vi "rename tag writer or reader.vi"(6 "new channel":refnum<class "TBM channel.lvclass">, 7 "owner ID":string, 8 "error in":errorcluster, 9 "old channel":refnum<class "TBM channel.lvclass">, 10 "tag descriptor":refnum<class "tag descriptor.lvclass">, 11 "engine configuration in":refnum<class "engine configuration.lvclass">) -> (0 "error out":errorcluster, 3 "engine configuration out":refnum<class "engine configuration.lvclass">)   [LabVIEW 2014, in "engine configuration.lvclass"]
uses:
  engine configuration.lvclass
  <vilib>/NI/Tag Bus/tag/tag descriptor.lvclass
  <vilib>/NI/Tag Bus Module Framework/channel/TBM channel.lvclass
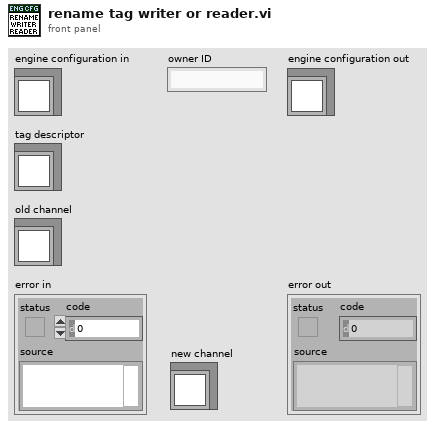
[diagram p1: front panel]
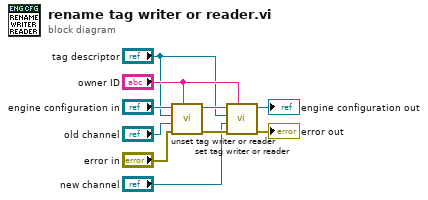
[diagram p0: block diagram]
diagram:
  n1 = call-dynamic "unset tag writer or reader.vi"("module GUID"="owner ID", "error in"="error in", "channel"="old channel", "tag descriptor"="tag descriptor", "engine configuration in"="engine configuration in") -> ("error out"=w9:errorcluster, "engine configuration out"=w10:refnum<class "engine configuration.lvclass">)  [unwired: 5 in]
  n2 = call-dynamic "set tag writer or reader.vi"("module GUID"="owner ID", "error in"=w9, "channel"="new channel", "tag descriptor"="tag descriptor", "engine configuration in"=w10) -> ("error out"=→"error out":errorcluster, "engine configuration out"=→"engine configuration out":refnum<class "engine configuration.lvclass">)  [unwired: 5 in]
